vi "TestDIO.vi"() -> ()   [LabVIEW 2021]
uses:
  Device Channels/Dependencies/DIO-Channel.lvlibp/Channels/DIO-Channel/DIO_Channel_class/DIO_Channel.lvclass
  Generic Channel/Channel.lvlib
  Device Channels/Dependencies/DIO-Channel.lvlibp
  Generic Channel/Channel/Channel_class/Channel.lvclass
  Device Channels/Dependencies/DIO-Channel.lvlibp/Generic Channel/Channel/Channel_class/Channel.lvclass
panel:
  in  "Output":bool
  out "Input 2":bool
  out "Success":bool
  in  "stop":bool
  out "Input":bool
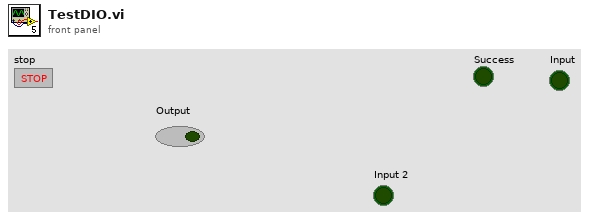
[diagram p1: front panel]
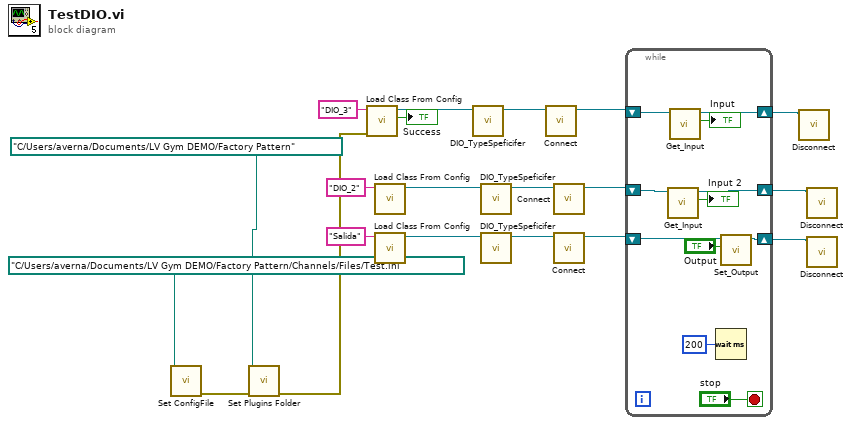
[diagram p0: block diagram]
diagram:
  n1 = call "Set ConfigFile.vi"("Plugins Folder"=path "C:/Users/averna/Documents/LV Gym DEMO/Factory Pattern/Channels/Files/Test.ini" ("Config File")) -> ("error out"=w19:errorcluster)  [unwired: 10 in]
  n2 = call "Set Plugins Folder.vi"("error in (no error)"=w19, "Config File"=path "C:/Users/averna/Documents/LV Gym DEMO/Factory Pattern" ("Plugins Folder")) -> ("error out"=w16:errorcluster)  [unwired: 9 in]
  n3 = call "Load Class From Config.vi"("error in (no error)"=w16, "Name"="DIO_3") -> ("Success"=→"Success":bool, "Channel"=w12:refnum<class "Channel.lvclass">)  [unwired: 7 in, 1 out]
  n4 = call "Load Class From Config.vi"("Name"="DIO_2") -> ("Channel"=w9:refnum<class "Channel.lvclass">)  [unwired: 8 in, 2 out]
  n5 = call "Load Class From Config.vi"("Name"="Salida") -> ("Channel"=w2:refnum<class "Channel.lvclass">)  [unwired: 8 in, 2 out]
  n6 = call "DIO_TypeSpeficifer.vi"("Channel"=w12) -> ("Type_Channel"=w11:refnum<class "DIO_Channel.lvclass">)  [unwired: 9 in, 1 out]
  n7 = call "DIO_TypeSpeficifer.vi"("Channel"=w9) -> ("Type_Channel"=w10:refnum<class "DIO_Channel.lvclass">)  [unwired: 9 in, 1 out]
  n8 = call "DIO_TypeSpeficifer.vi"("Channel"=w2) -> ("Type_Channel"=w1:refnum<class "DIO_Channel.lvclass">)  [unwired: 9 in, 1 out]
  n9 = call-dynamic "Connect.vi"("object in"=w11) -> ("object out"=w13:refnum<class "DIO_Channel.lvclass">)  [unwired: 8 in, 2 out]
  n10 = call-dynamic "Connect.vi"("object in"=w10) -> ("object out"=w8:refnum<class "DIO_Channel.lvclass">)  [unwired: 8 in, 2 out]
  n11 = call-dynamic "Connect.vi"("object in"=w1) -> ("object out"=w3:refnum<class "DIO_Channel.lvclass">)  [unwired: 8 in, 2 out]
  n12 = while {
    shift-right: [w30] -> w15
    shift-left: w13 -> [w31]
    shift-right: [w25] -> w7
    shift-left: w8 -> [w24]
    shift-right: [w22] -> w4
    shift-left: w3 -> [w23]
    stop <- "stop" stop-if-true
    n13 = call-dynamic "Get_Input.vi"("object in"=w24) -> ("Input"=→"Input 2":bool, "object out"=w25:refnum<class "DIO_Channel.lvclass">)  [unwired: 8 in, 1 out]
    n14 = call-dynamic "Get_Input.vi"("object in"=w31) -> ("Input"=→"Input":bool, "object out"=w30:refnum<class "DIO_Channel.lvclass">)  [unwired: 8 in, 1 out]
    n15 = Wait (ms)(milliseconds to wait=u32 200) -> ()  [unwired: 1 out]
    n16 = call-dynamic "Set_Output.vi"("Output"="Output", "object in"=w23) -> ("object out"=w22:refnum<class "DIO_Channel.lvclass">)  [unwired: 8 in, 1 out]
  }
  n17 = call-dynamic "Disconnect.vi"("object in"=w15) -> ()  [unwired: 9 in, 2 out]
  n18 = call-dynamic "Disconnect.vi"("object in"=w7) -> ()  [unwired: 9 in, 2 out]
  n19 = call-dynamic "Disconnect.vi"("object in"=w4) -> ()  [unwired: 9 in, 2 out]
